vi "Main_RT_V1.vi"() -> ()   [LabVIEW 2018]
uses:
  enum_bras.ctl
  <vilib>/Platform/TimedLoop/XDataNode/timing_clust.ctl
  <vilib>/Platform/TimedLoop/XDataNode/nitl_modes.ctl
  <vilib>/Platform/TimedLoop/XDataNode/wakeup.ctl
  enum_RT_Seaux.ctl
  enum_RT_Virage.ctl
  enum_RT_recule.ctl
  enum_RT_trieur_Balles.ctl
  enum_RT_lanceur.ctl
  <vilib>/Platform/TimedLoop/XDataNode/XDataNode.xnode
  <vilib>/Platform/TimedLoop/XDataNode/XDNodeRunTimeDep.lvlib
panel:
  out "Sceaux":bool
  out "Lanceur de balles":bool
  out "Virage 4":bool
  out "Virage 3":bool
  out "Clapets 2":bool
  out "Trieur de Balles":bool
  out "Reculer":bool
  out "Virage 2":bool
  out "Virage 1":bool
  out "Clapets 1":bool
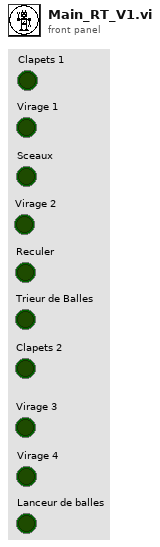
[diagram p1: front panel]
types:
  T1 = typedef "enum_bras.ctl" = enum16{"Depart Bras", "Clapet Bras", "Inactif Bras", "Seaux Bras"}
  T2 = typedef "XDNodeRunTimeDep.lvlib/timing_clust.ctl" = cluster{"Expected End [f-1]":u64, "Actual End [f-1]":u64, "Finished Late? [f-1]":bool, "Expected End [i-1]":u64, "Actual End [i-1]":u64, "Finished Late? [i-1]":bool, "Expected Start [i]":u64, "Actual Start [i]":u64, "Expected Start [f]":u64, "Actual Start [f]":u64, "Source Name":string, "Structure Name":string, "Period":i64, "Deadline":i64, "Offset":i64, "Start":i64, "Priority":i32, "Timeout":i32, "Mode":T3, "Wakeup Reason":T4, "Error":errorcluster, "Source Type":string, "Secondary Source Type":string, "Global End Time":u64, "Global Start Time":u64, "Frame Duration":u64, "Iteration Duration":u64, "Assigned CPU":i32, "I/O Scan Engine Mode":u32}
  T3 = typedef "XDNodeRunTimeDep.lvlib/nitl_modes.ctl" = enum32{"No Change", "Process missed periods, maintain original phase", "Discard missed periods, maintain original phase", "Process missed periods, ignore original phase", "Discard missed periods, ignore original phase"}
  T4 = typedef "XDNodeRunTimeDep.lvlib/wakeup.ctl" = enum32{"Normal", "Aborted", "Asynchronous wakeup", "Timing source error", "Timed loop error", "Timeout"}
  T5 = typedef "enum_RT_Seaux.ctl" = enum16{"Avancé 1", "Ready to Start", "Stop moteur", "Bras Inactif 1", "Frappe sceau", "Bras Inactif 2", "Avancé 2"}
  T6 = typedef "enum_RT_Virage.ctl" = enum16{"Avancer", "STOP", "Lacher Ligne", "Tourner"}
  T7 = typedef "enum_RT_recule.ctl" = enum16{"Avancer", "Reculer", "STOP"}
  T8 = typedef "enum_RT_trieur_Balles.ctl" = enum16{"Initialisation", "Couleur", "Rotation1", "Rotation2", "Ouverture", "Fermeture"}
  T9 = typedef "enum_RT_lanceur.ctl" = enum16{"eloignement", "arret_robot", "moteur_lanceur", "distributeur", "arret_distributeur_lanceur"}
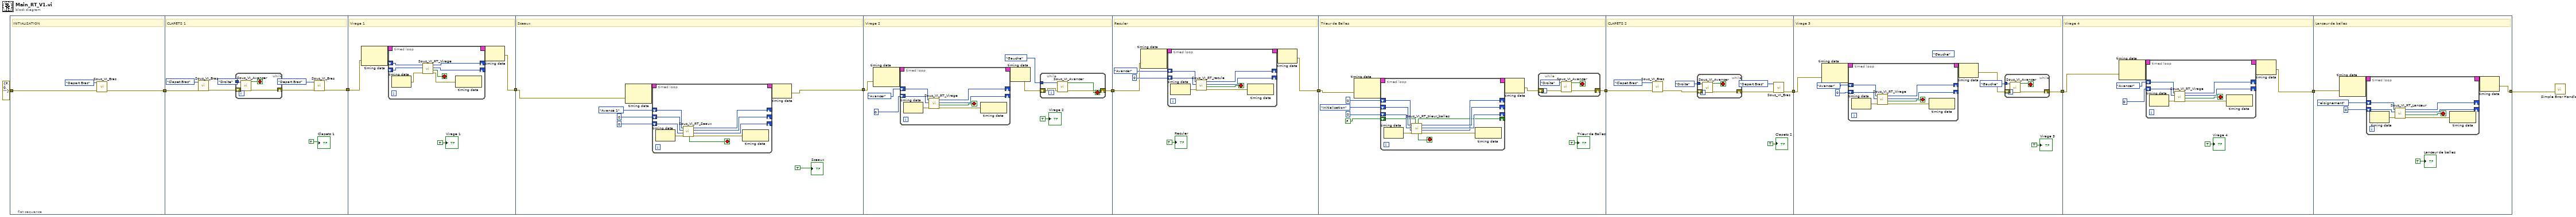
[diagram p0: block diagram]
diagram:
  n1 = flat-sequence {
    tunnel: errorcluster {"status"=FALSE, "code"=0, "source"=""} ("error in (no error)") -> [w15]
    tunnel: [w14] -> w9
    tunnel: [w18] -> w10
    tunnel: w9 -> [w22]
    tunnel: w10 -> [w29]
    tunnel: [w28] -> w2
    tunnel: w2 -> [w50]
    tunnel: [w51] -> w1
    tunnel: [w85] -> w8
    tunnel: w1 -> [w81]
    tunnel: [w107] -> w11
    tunnel: w8 -> [w108]
    tunnel: w11 -> [w131]
    tunnel: [w140] -> w7
    tunnel: w7 -> [w171]
    tunnel: [w167] -> w6
    tunnel: w6 -> [w179]
    tunnel: [w185] -> w5
    tunnel: w5 -> [w208]
    tunnel: [w209] -> w4
    tunnel: w4 -> [w233]
    tunnel: [w232] -> w3
    frame #0 {
      # "INITIALISATION"
      n2 = call "Sous_VI_Bras.vi"("error in (no error)"=w15, "Enum bras"=enum_bras."Depart Bras") -> ("error out"=w14:errorcluster)  [unwired: 9 in]
    }
    frame #1 {
      # "CLAPETS 1"
      n3 = call "Sous_VI_Bras.vi"("error in (no error)"=w22, "Enum bras"=enum_bras."Clapet Bras") -> ("error out"=w17:errorcluster)  [unwired: 9 in]
      n4 = while {
        tunnel: enum16{"Droite", "Gauche"}."Droite" ("Énum") -> [w27]
        shift-right: [w26] -> w19
        shift-left: w17 -> [w25]
        stop <- w24 stop-if-true
        n5 = call "Sous_VI_Avancer.vi"("error in (no error)"=w25, "Énum"=w27) -> ("error out"=w26:errorcluster, "Info de fin de Parcours"=w24:bool)  [unwired: 7 in, 1 out]
      }
      n6 = call "Sous_VI_Bras.vi"("error in (no error)"=w19, "Enum bras"=enum_bras."Depart Bras") -> ("error out"=w18:errorcluster)  [unwired: 9 in]
      "Clapets 1" <- TRUE ("Booléen")
    }
    frame #2 {
      # "Virage 1"
      n7 = node-c288(w29) -> (w31:T2)  [unwired: 1 in]
      n8 = timed-loop {
        timing: w31 -> [_]
        timing-out: [_] -> w30
        shift-right: [w37] -> _
        shift-left: _ -> [w35]
        shift-right: [w36] -> _
        shift-left: _ -> [w34]
        stop <- w33 stop-if-true
        n9 = node-c288() -> (w39:errorcluster)  [unwired: 1 in]
        n10 = call "Sous_VI_RT_Virage.vi"("Erreur in"=w39, "Compteur IN"=w34, "Etat IN"=w35) -> ("Erreur out"=w38:errorcluster, "Information de fin de process"=w33:bool, "Compteur OUT"=w36:i32, "Etat OUT"=w37:T6)  [unwired: 4 in, 1 out]
        n11 = node-c288(w38) -> ()  [unwired: 1 out]
      }
      n12 = node-c288(w30) -> (w28:errorcluster)
      "Virage 1" <- TRUE ("Booléen")
    }
    frame #3 {
      # "Sceaux"
      n13 = node-c288(w50) -> (w57:T2)  [unwired: 1 in]
      n14 = timed-loop {
        timing: w57 -> [_]
        timing-out: [_] -> w56
        shift-right: [w63] -> _
        shift-left: 0 -> [w66]
        shift-right: [w58] -> _
        shift-left: enum_RT_Seaux."Avancé 1" ("Etat IN") -> [w59]
        shift-right: [w62] -> _
        shift-left: 0 -> [w65]
        stop <- w64 stop-if-true
        n15 = node-c288() -> (w61:errorcluster)  [unwired: 1 in]
        n16 = call "Sous_VI_RT_Seaux.vi"("Erreur IN"=w61, "Nombre Sceau IN"=w65, "Compteur IN"=w66, "Etat IN"=w59) -> ("Erreur OUT"=w60:errorcluster, "Nombre Sceau OUT"=w62:i32, "Compteur OUT"=w63:i32, "Etat OUT"=w58:T5, "Indicateur de fin de process"=w64:bool)  [unwired: 2 in, 1 out]
        n17 = node-c288(w60) -> ()  [unwired: 1 out]
      }
      n18 = node-c288(w56) -> (w51:errorcluster)
      "Sceaux" <- TRUE ("Booléen")
    }
    frame #4 {
      # "Virage 2"
      n19 = node-c288(w81) -> (w83:T2)  [unwired: 1 in]
      n20 = timed-loop {
        timing: w83 -> [_]
        timing-out: [_] -> w82
        shift-right: [w90] -> _
        shift-left: enum_RT_Virage."Avancer" ("Etat OUT") -> [w88]
        shift-right: [w89] -> _
        shift-left: 0 ("Compteur OUT") -> [w87]
        stop <- w86 stop-if-true
        n21 = node-c288() -> (w92:errorcluster)  [unwired: 1 in]
        n22 = call "Sous_VI_RT_Virage.vi"("Erreur in"=w92, "Compteur IN"=w87, "Etat IN"=w88) -> ("Erreur out"=w91:errorcluster, "Information de fin de process"=w86:bool, "Compteur OUT"=w89:i32, "Etat OUT"=w90:T6)  [unwired: 4 in, 1 out]
        n23 = node-c288(w91) -> ()  [unwired: 1 out]
      }
      n24 = node-c288(w82) -> (w80:errorcluster)
      n25 = while {
        tunnel: enum16{"Droite", "Gauche"}."Gauche" ("Énum") -> [w106]
        shift-right: [w104] -> w85
        shift-left: w80 -> [w105]
        stop <- w103 stop-if-true
        n26 = call "Sous_VI_Avancer.vi"("error in (no error)"=w105, "Énum"=w106) -> ("error out"=w104:errorcluster, "Info de fin de Parcours"=w103:bool)  [unwired: 7 in, 1 out]
      }
      "Virage 2" <- TRUE ("Booléen")
    }
    frame #5 {
      # "Reculer"
      n27 = node-c288(w108) -> (w112:T2)  [unwired: 1 in]
      n28 = timed-loop {
        timing: w112 -> [_]
        timing-out: [_] -> w111
        shift-right: [w117] -> _
        shift-left: 0 -> [w116]
        shift-right: [w114] -> _
        shift-left: enum_RT_recule."Avancer" ("Etat OUT") -> [w115]
        stop <- w118 stop-if-true
        n29 = node-c288() -> (w120:errorcluster)  [unwired: 1 in]
        n30 = call "Sous_VI_RT_recule.vi"("Erreur IN"=w120, "Compteur IN"=w116, "Etat IN"=w115) -> ("Erreur OUT"=w119:errorcluster, "Indicateur fin de process"=w118:bool, "Compteur OUT"=w117:i32, "Etat OUT"=w114:T7)  [unwired: 4 in, 1 out]
        n31 = node-c288(w119) -> ()  [unwired: 1 out]
      }
      n32 = node-c288(w111) -> (w107:errorcluster)
      "Reculer" <- TRUE ("Booléen")
    }
    frame #6 {
      # "Trieur de Balles"
      n33 = node-c288(w131) -> (w138:T2)  [unwired: 1 in]
      n34 = timed-loop {
        timing: w138 -> [_]
        timing-out: [_] -> w137
        shift-right: [w148] -> _
        shift-left: 0 -> [w149]
        shift-right: [w146] -> _
        shift-left: 0 -> [w147]
        shift-right: [w150] -> _
        shift-left: enum_RT_trieur_Balles."Initialisation" ("Etat IN") -> [w151]
        shift-right: [w141] -> _
        shift-left: FALSE -> [w142]
        stop <- w145 stop-if-true
        n35 = node-c288() -> (w144:errorcluster)  [unwired: 1 in]
        n36 = call "Sous_VI_RT_trieur_balles.vi"("Détection couleur IN"=w142, "error in (no error)"=w144, "Nombre Balle IN"=w147, "Comteur IN"=w149, "Etat IN"=w151) -> ("error out"=w143:errorcluster, "Nombre Balle OUT"=w146:i32, "Comteur OUT"=w148:i32, "Etat OUT"=w150:T8, "Indicateur de fin de process"=w145:bool, "Détection couleur OUT"=w141:bool)  [unwired: 1 in]
        n37 = node-c288(w143) -> ()  [unwired: 1 out]
      }
      n38 = node-c288(w137) -> (w132:errorcluster)
      n39 = while {
        shift-right: [w163] -> w140
        shift-left: w132 -> [w164]
        stop <- w162 stop-if-true
        n40 = call "Sous_VI_Avancer.vi"("error in (no error)"=w164, "Énum"=enum16{"Droite", "Gauche"}."Droite") -> ("error out"=w163:errorcluster, "Info de fin de Parcours"=w162:bool)  [unwired: 7 in, 1 out]
      }
      "Trieur de Balles" <- TRUE ("Booléen")
    }
    frame #7 {
      # "CLAPETS 2"
      n41 = call "Sous_VI_Bras.vi"("error in (no error)"=w171, "Enum bras"=enum_bras."Clapet Bras") -> ("error out"=w170:errorcluster)  [unwired: 9 in]
      n42 = while {
        tunnel: enum16{"Droite", "Gauche"}."Droite" ("Énum") -> [w177]
        shift-right: [w175] -> w168
        shift-left: w170 -> [w176]
        stop <- w174 stop-if-true
        n43 = call "Sous_VI_Avancer.vi"("error in (no error)"=w176, "Énum"=w177) -> ("error out"=w175:errorcluster, "Info de fin de Parcours"=w174:bool)  [unwired: 7 in, 1 out]
      }
      n44 = call "Sous_VI_Bras.vi"("error in (no error)"=w168, "Enum bras"=enum_bras."Depart Bras") -> ("error out"=w167:errorcluster)  [unwired: 9 in]
      "Clapets 2" <- TRUE ("Booléen")
    }
    frame #8 {
      (unwired) enum16{"Droite", "Gauche"}."Gauche" ("Énum")
      # "Virage 3"
      n45 = node-c288(w179) -> (w183:T2)  [unwired: 1 in]
      n46 = timed-loop {
        timing: w183 -> [_]
        timing-out: [_] -> w182
        shift-right: [w191] -> _
        shift-left: enum_RT_Virage."Avancer" ("Etat OUT") -> [w189]
        shift-right: [w190] -> _
        shift-left: 0 ("Compteur OUT") -> [w188]
        stop <- w187 stop-if-true
        n47 = node-c288() -> (w193:errorcluster)  [unwired: 1 in]
        n48 = call "Sous_VI_RT_Virage.vi"("Erreur in"=w193, "Compteur IN"=w188, "Etat IN"=w189) -> ("Erreur out"=w192:errorcluster, "Information de fin de process"=w187:bool, "Compteur OUT"=w190:i32, "Etat OUT"=w191:T6)  [unwired: 4 in, 1 out]
        n49 = node-c288(w192) -> ()  [unwired: 1 out]
      }
      n50 = node-c288(w182) -> (w178:errorcluster)
      n51 = while {
        tunnel: enum16{"Droite", "Gauche"}."Gauche" ("Énum") -> [w207]
        shift-right: [w205] -> w185
        shift-left: w178 -> [w206]
        stop <- w204 stop-if-true
        n52 = call "Sous_VI_Avancer.vi"("error in (no error)"=w206, "Énum"=w207) -> ("error out"=w205:errorcluster, "Info de fin de Parcours"=w204:bool)  [unwired: 7 in, 1 out]
      }
      "Virage 3" <- TRUE ("Booléen")
    }
    frame #9 {
      # "Virage 4"
      n53 = node-c288(w208) -> (w213:T2)  [unwired: 1 in]
      n54 = timed-loop {
        timing: w213 -> [_]
        timing-out: [_] -> w212
        shift-right: [w219] -> _
        shift-left: enum_RT_Virage."Avancer" ("Etat OUT") -> [w217]
        shift-right: [w218] -> _
        shift-left: 0 ("Compteur OUT") -> [w216]
        stop <- w215 stop-if-true
        n55 = node-c288() -> (w221:errorcluster)  [unwired: 1 in]
        n56 = call "Sous_VI_RT_Virage.vi"("Erreur in"=w221, "Compteur IN"=w216, "Etat IN"=w217) -> ("Erreur out"=w220:errorcluster, "Information de fin de process"=w215:bool, "Compteur OUT"=w218:i32, "Etat OUT"=w219:T6)  [unwired: 4 in, 1 out]
        n57 = node-c288(w220) -> ()  [unwired: 1 out]
      }
      n58 = node-c288(w212) -> (w209:errorcluster)
      "Virage 4" <- TRUE ("Booléen")
    }
    frame #10 {
      # "Lanceur de balles"
      n59 = node-c288(w233) -> (w237:T2)  [unwired: 1 in]
      n60 = timed-loop {
        timing: w237 -> [_]
        timing-out: [_] -> w236
        shift-right: [w241] -> _
        shift-left: enum_RT_lanceur."eloignement" ("enum_out") -> [w242]
        shift-right: [w239] -> _
        shift-left: 0 ("Compteur OUT") -> [w240]
        stop <- w245 stop-if-true
        n61 = node-c288() -> (w244:errorcluster)  [unwired: 1 in]
        n62 = call "Sous_VI_RT_Lanceur.vi"("Erreur_in"=w244, "cpt_in"=w240, "enum_in"=w242) -> ("Erreur_out"=w243:errorcluster, "vi_fini"=w245:bool, "cpt_out"=w239:i32, "enum_out"=w241:T9)  [unwired: 4 in, 1 out]
        n63 = node-c288(w243) -> ()  [unwired: 1 out]
      }
      n64 = node-c288(w236) -> (w232:errorcluster)
      "Lanceur de balles" <- TRUE ("Booléen")
    }
  }
  n65 = call <vilib>:"Simple Error Handler.vi"("error in (no error)"=w3) -> ()  [unwired: 4 in, 5 out]
